vi "Create Runtime.vi"(8 "error in (no error)":errorcluster, 11 "CIFChannels in":refnum<class "CIFChannels.lvclass">) -> (0 "error out":errorcluster, 3 "CIFChannels out":refnum<class "CIFChannels.lvclass">)   [LabVIEW 2021, in "CIFChannels.lvclass"]
doc: "To support channels that get reconfigured for different sizes or queue depths, the publisher create can register but not actually create the underlying FIFO. Instead the creation can be delayed and can be created at run-time. This function is called for each channel on prepare and when a subscriber connects."
uses:
  CIFChannels.lvclass
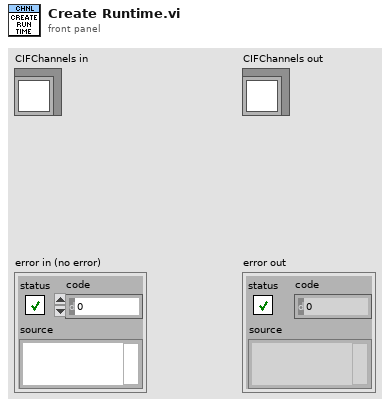
[diagram p1: front panel]
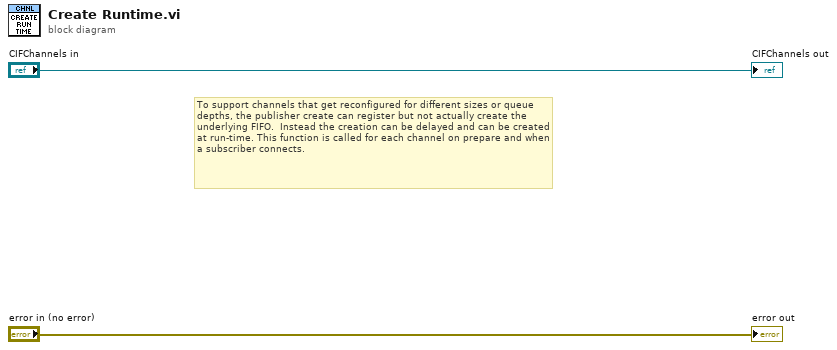
[diagram p0: block diagram]
diagram:
  # "To support channels that get reconfigured for different sizes or queue depths, the publisher create can register but not actually create the underlying FIFO.  Instead the creation can be delayed and can be created at run-time. This function is called for each channel on prepare and when a subscriber connects."
  "error out" <- "error in (no error)"
  "CIFChannels out" <- "CIFChannels in"
